vi "NewMain.vi"() -> ()   [LabVIEW 2016, in "13.03 Robot.lvrbt"]
uses:
  13.03 Robot.lvrbt
  <vilib>/NXT/Block Support/NXT_OutputPort.ctl
  <vilib>/NXT/Subs/ColorSensorColors.ctl
  <vilib>/NXT/Block Support/NXT_InputPort.ctl
  <vilib>/NXT/Dual Mode Library/Display/drawText.vi
  <vilib>/NXT/Dual Mode Library/Display/drawNumber.vi
panel:
  out "isHeavy":bool
  in  "ColorH":T1=enum."Blue"
  in  "ColorL":T1=enum."Blue"
  in  "Bin Sense Threshold":dbl=10.0
  in  "Turn Power":dbl=30.0
  in  "Movement Power":dbl=30.0
  in  "Black Threshold":sgl=20.0
  in  "Motor IDs":cluster{"Motors":T2, "Motors 2":T2}={"Motors"=0, "Motors 2"=1} {"Motors 2" items=["Port A", "Port B", "Port C", "Port D"]; "Motors" items=["Port A", "Port B", "Port C", "Port D"]}
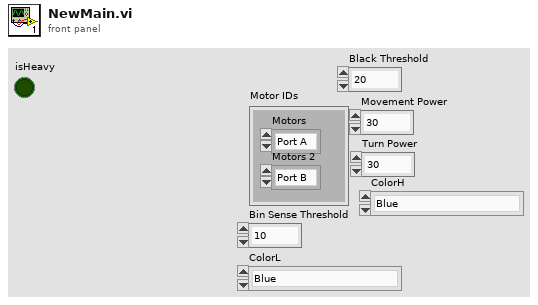
[diagram p1: front panel]
types:
  T1 = typedef "ColorSensorColors.ctl" = enum16{"No Color", "Black", "Blue", "Green", "Yellow", "Red", "White", "Brown"}
  T2 = typedef "NXT_OutputPort.ctl" = u8
  T3 = typedef "NXT_InputPort.ctl" = u32
  T4 = typedef "LVHSConnector.ctl" = refnum<class "BrickReference.lvclass">
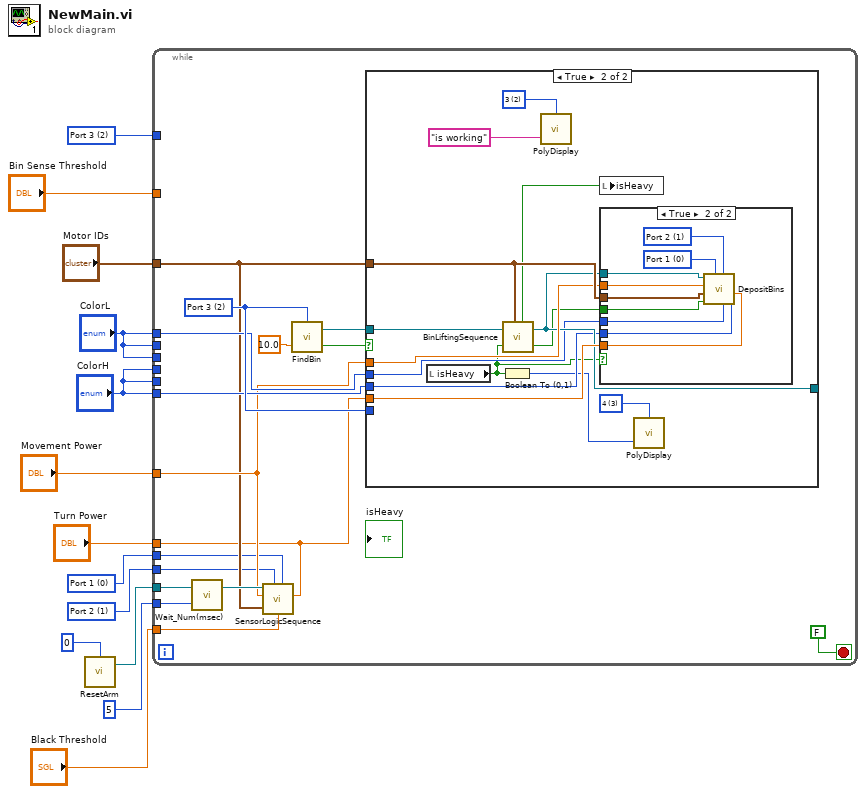
[diagram p0: block diagram]
diagram:
  w8 = T3 2 items=["Port 1", "Port 2", "Port 3", "Port 4"] ("Port")
  w11 = T3 0 items=["Port 1", "Port 2", "Port 3", "Port 4"] ("Port (Port 1)")
  w13 = T3 1 items=["Port 1", "Port 2", "Port 3", "Port 4"] ("Port (Port 1)")
  n1 = call "ResetArm.vi"("ResetTo"=0) -> ("NXT/EV3 OUT"=w4:T4)  [unwired: 2 in]
  n2 = while {
    tunnel: w13 -> [w15]
    tunnel: u32 5 ("Time (100 msec)") -> [w29]
    tunnel: w11 -> [w16]
    tunnel: "Motor IDs" -> [w17]
    tunnel: "Black Threshold" -> [w27]
    tunnel: w8 -> [_]
    tunnel: "Movement Power" -> [w18]
    tunnel: "Turn Power" -> [w14]
    tunnel: "Bin Sense Threshold" -> [_]
    tunnel: "ColorH" -> [_]
    tunnel: "ColorL" -> [_]
    tunnel: w4 -> [w21]
    tunnel: "ColorL" -> [w20]
    tunnel: "ColorH" -> [w19]
    tunnel: "ColorL" -> [_]
    tunnel: "ColorH" -> [_]
    stop <- FALSE stop-if-true
    w22 = T3 2 items=["Port 1", "Port 2", "Port 3", "Port 4"] ("Port")
    n3 = call <vilib>:"Wait_Num(msec).vi"("Time (100 msec)"=w29, "NXT/EV3"=w21) -> ("NXT/EV3"=w26:T4)  [unwired: 2 in]
    n4 = call "SensorLogicSequence.vi"("Turn Power"=w14, "Port 2"=w16, "Port 1"=w15, "Movement Power"=w18, "NXT/EV3 IN"=w26, "Black Threshold"=w27, "Motor IDs"=w17) -> ()  [unwired: 1 in, 1 out]
    n5 = call "FindBin.vi"("Threshold"=10.0, "Port"=w22) -> ("Out"=w24:bool, "NXT/EV3 OUT"=w23:T4)  [unwired: 1 in]
    n6 = case shown="True" w24 {
      tunnel: w23 -> [w30 w44]
      tunnel: w17 -> [_ w43]
      tunnel: w22 -> [_ _]
      tunnel: [w30 w40] -> _
      tunnel: w18 -> [_ w42]
      tunnel: w14 -> [_ w41]
      tunnel: w20 -> [_ w36]
      tunnel: w19 -> [_ w35]
      frame False {
      }
      frame True {
        w33 = i16 3 items=["1", "2", "3", "4", "5", "6", "7", "8", "9", "10", "11", "12"] ("Line")
        w38 = i16 2 items=["1", "2", "3", "4", "5", "6", "7", "8", "9", "10", "11", "12"] ("Line")
        n7 = local read "isHeavy"() -> (w31:bool)
        n8 = Boolean To (0,1)(Boolean=w31) -> (0, 1=w34:i16)
        n9 = call "BinLiftingSequence.vi"("isAlreadyPickedUp"=w31, "NXT/EV3 IN"=w44, "Motor IDs"=w43) -> ("IsHeavy"=w39:bool, "alreadyPickedUp"=w32:bool, "NXT/EV3 OUT"=w40:T4)
        n10 = call-poly <vilib>:"PolyDisplay.vi"("Text"="is working", "Line"=w38) -> ()  [unwired: 2 in, 1 out]
        n11 = local write "isHeavy"(w32) -> ()
        n12 = case shown="True" w31 {
          tunnel: w43 -> [_ w48]
          tunnel: w42 -> [_ w50]
          tunnel: w41 -> [_ w49]
          tunnel: w40 -> [_ w51]
          tunnel: w39 -> [_ w47]
          tunnel: w36 -> [_ w46]
          tunnel: w35 -> [_ w45]
          frame False {
          }
          frame True {
            w53 = T3 1 items=["Port 1", "Port 2", "Port 3", "Port 4"] ("Port 2")
            w52 = T3 0 items=["Port 1", "Port 2", "Port 3", "Port 4"] ("Port 1")
            n13 = call "DepositBins.vi"("Port 2"=w53, "Port 1"=w52, "NXT/EV3 IN"=w51, "Movement Power"=w50, "Turn Power"=w49, "Motor IDs"=w48, "ColorH"=w45, "ColorL"=w46, "isHeavy"=w47) -> ()  [unwired: 2 out]
          }
        }
        n14 = call-poly <vilib>:"PolyDisplay.vi"("number"=w34, "Line"=w33) -> ()  [unwired: 2 in, 1 out]
      }
    }
  }
